vi "FuncVI2-_Exec.vi"(4 "Caller CSE RefNum":T1, 5 "InstanceRef":T3, 9 "arg list":T2[](array[typedef]) {"num" format="%.2f"}) -> (0 "error out":bool, 3 "result":T2 {"num" format="%.2f"})   [LabVIEW 2021]
doc: "::: CalcExpress Toolkit :::\nCopyright (c) 2000-2026 Konstantin Shifershteyn. All rights reserved."
uses:
  cetypes.llb/CalcExpress Function Argument Info.ctl
  cetypes.llb/CalcExpress Instance RefNum.ctl
  cse.llb/CSE Instance RefNum.ctl
panel:
  in  "max arg num":i32=1
  in  "min arg num":i32=1
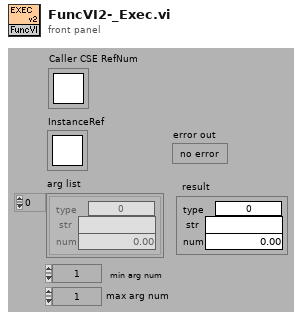
[diagram p1: front panel]
types:
  T1 = typedef "CSE Instance RefNum.ctl" = refnum<k1>
  T2 = typedef "CalcExpress Function Argument Info.ctl" = cluster{"type":u32, "str":string, "num":dbl}
  T3 = typedef "CalcExpress Instance RefNum.ctl" = refnum<k1>
  T4 = enum32{"String", "DBL Number", "identifier", "1D Array of DBL", "2D Array of DBL", "CDB Number", "1D Array of CDB", "2D Array of CDB", "1D Array of String", "2D Array of String", "Unknown data type"}
  T5 = typedef "CSE Callback VI RefNum.ctl" = refnum<vi>
  T6 = typedef "VarMan Variable Context Handle.ctl" = i32
  T7 = cluster{"type: use this constant to specify a predefined type code":enum32{"String", "DBL Number", "identifier", "1D Array of DBL", "2D Array of DBL", "CDB Number", "1D Array of CDB", "2D Array of CDB", "1D Array of String", "2D Array of String", "Unknown data type"}, string, "return value":dbl}
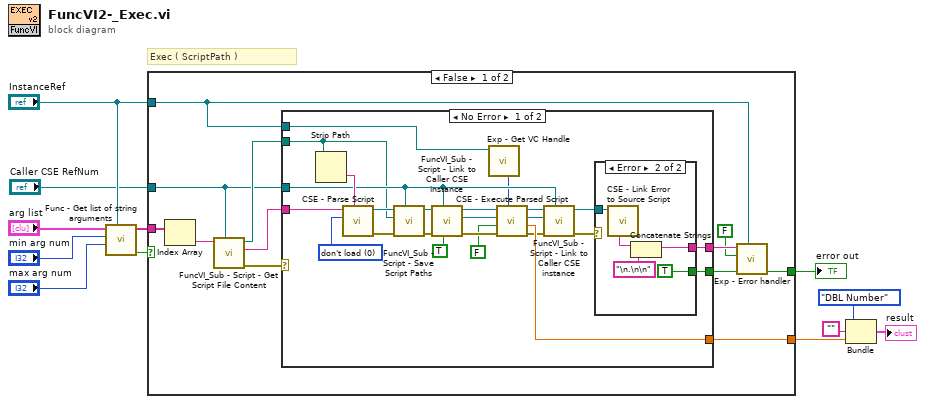
[diagram p0: block diagram]
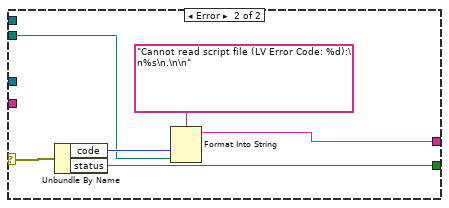
[diagram p3: hidden frame]
diagram:
  # "Exec ( ScriptPath )"
  n1 = call "Func - Get list of string arguments.vi"("InstanceRef"="InstanceRef", "max arg num"="max arg num", "min arg num"="min arg num", "arg list"="arg list") -> ("error out"=w7:bool, "val list"=w8:string[])  [unwired: 4 in]
  n2 = case shown="False" w7 {
    selector: w7 -> [_ w60]
    tunnel: "InstanceRef" -> [w19 _]
    tunnel: w8 -> [w18 _]
    tunnel: [w23 w60] -> w6
    tunnel: [w24 _] -> w2
    tunnel: "Caller CSE RefNum" -> [w13 _]
    frame False {
      n3 = Index Array(array=w18) -> (element=w16:string)  [unwired: 1 in]
      n4 = call "FuncVI_Sub - Script - Get Script File Content.vi"("Caller CSE RefNum"=w13, "Script name"=w16) -> ("error out"=w17:errorcluster, "Script body"=w15:string, "Script Path"=w14:path)  [unwired: 7 in]
      n5 = case shown="No Error" w17 {
        selector: w17 -> [_ w59]
        tunnel: w15 -> [w48 _]
        tunnel: [w47 _] -> w24
        tunnel: [w45 w57] -> w22
        tunnel: w14 -> [w29 w54]
        tunnel: [w46 w56] -> w21
        tunnel: w13 -> [w30 _]
        tunnel: w19 -> [w26 _]
        frame No Error {
          w44 = u32 0 items=["don't load", "load", "load & test"] ("load FuncVIs")
          n6 = Strip Path(path=w29) -> (name=w43:string)  [unwired: 1 out]
          n7 = call "CSE - Parse Script.vi"("Script name"=w43, "load FuncVIs"=w44, "Script"=w48) -> ("error out"=w34:errorcluster, "CSE RefNum"=w31:T1)  [unwired: 4 in, 3 out]
          n8 = call "FuncVI_Sub - Script - Save Script Paths.vi"("Caller CSE RefNum"=w30, "error in"=w34, "Script File Path"=w29, "CSE RefNum"=w31) -> ("error out"=w33:errorcluster, "dup CSE RefNum"=w32:T1)  [unwired: 6 in]
          n9 = call "FuncVI_Sub - Script - Link to Caller CSE instance.vi"("Link(T)/Delink(F)"=TRUE, "Caller CSE RefNum"=w30, "error in"=w33, "CSE RefNum"=w32) -> ("error out"=w37:errorcluster, "Callback VI RefNum out"=w38:T5, "dup CSE RefNum"=w39:T1)  [unwired: 5 in]
          n10 = call "Exp - Get VC Handle.vi"("InstanceRef"=w26) -> ("VC Handle"=w27:T6)  [unwired: 5 in, 3 out]
          n11 = call "CSE - Execute Parsed Script.vi"("VC Handle"=w27, "error in"=w37, "Close FuncVI Refs (T)"=FALSE, "Callback VI RefNum"=w38, "CSE RefNum"=w39) -> ("error out"=w35:errorcluster, "return value"=w47:dbl, "dup Callback VI RefNum"=w40:T5, "dup CSE RefNum"=w42:T1)  [unwired: 2 in, 1 out]
          n12 = call "FuncVI_Sub - Script - Link to Caller CSE instance.vi"("Caller CSE RefNum"=w30, "error in"=w35, "Callback VI RefNum"=w40, "CSE RefNum"=w42) -> ("error out"=w28:errorcluster, "dup CSE RefNum"=w41:T1)  [unwired: 5 in, 1 out]
          n13 = case shown="Error" w28 {
            tunnel: w41 -> [_ w53]
            tunnel: [_ TRUE] -> w45
            tunnel: [_ w49] -> w46
            frame No Error {
            }
            frame Error {
              n14 = call "CSE - Link Error to Source Script.vi"("CSE RefNum"=w53) -> ("Error Message"=w51:string)  [unwired: 4 in, 6 out]
              n15 = Concatenate Strings(w51, "\n.\n\n" ("string")) -> (w49:string)
            }
          }
        }
        frame Error {
          n16 = Unbundle By Name(w59) -> ("code"=w55:i32, "status"=w57:bool)
          n17 = Format Into String(format string="Cannot read script file (LV Error Code: %d):\n%s\n.\n\n", w55, w54) -> (resulting string=w56:string)  [unwired: 2 in, 1 out]
        }
      }
      n18 = call "Exp - Error handler.vi"("InstanceRef"=w19, "error in"=w22, "add FuncName (T)"=FALSE, "error message in"=w21) -> ("error out"=w23:bool)  [unwired: 5 in, 2 out]
    }
    frame True {
    }
  }
  "error out" <- w6
  n19 = Bundle("type: use this constant to specify a predefined type code"=T4."DBL Number", "", "return value"=w2) -> (→"result":T7)  [unwired: 1 in]
